vi "FuncVI-viRun.vi"(5 "InstanceRef":T2, 9 "arg list":T1[](array[typedef]) {"num" format="%.2f"}) -> (0 "error out":bool, 3 "result":T1 {"num" format="%.2f"})   [LabVIEW 2021]
doc: "::: CalcExpress Toolkit :::\nCopyright (c) 2000-2026 Konstantin Shifershteyn. All rights reserved."
uses:
  cetypes.llb/CalcExpress Function Argument Info.ctl
  cetypes.llb/CalcExpress Instance RefNum.ctl
panel:
  in  "max arg num":i32=1000
  in  "min arg num":i32=1
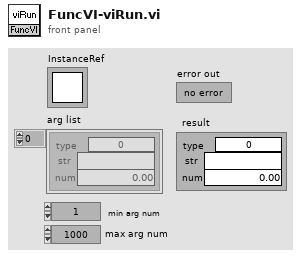
[diagram p1: front panel]
types:
  T1 = typedef "CalcExpress Function Argument Info.ctl" = cluster{"type":u32, "str":string, "num":dbl}
  T2 = typedef "CalcExpress Instance RefNum.ctl" = refnum<k1>
  T3 = enum32{"String", "DBL Number", "identifier", "1D Array of DBL", "2D Array of DBL", "CDB Number", "1D Array of CDB", "2D Array of CDB", "1D Array of String", "2D Array of String", "Unknown data type"}
  T4 = cluster{"index":i32, "data type":enum32{"String", "DBL Number", "identifier", "1D Array of DBL", "2D Array of DBL", "CDB Number", "1D Array of CDB", "2D Array of CDB", "1D Array of String", "2D Array of String", "Unknown data type"}, "default num":dbl, "default str":string}[]
  T5 = cluster{"use this constant to specify a predefined type":enum32{"String", "DBL Number", "identifier", "1D Array of DBL", "2D Array of DBL", "CDB Number", "1D Array of CDB", "2D Array of CDB", "1D Array of String", "2D Array of String", "Unknown data type"}, string, "code":i32}
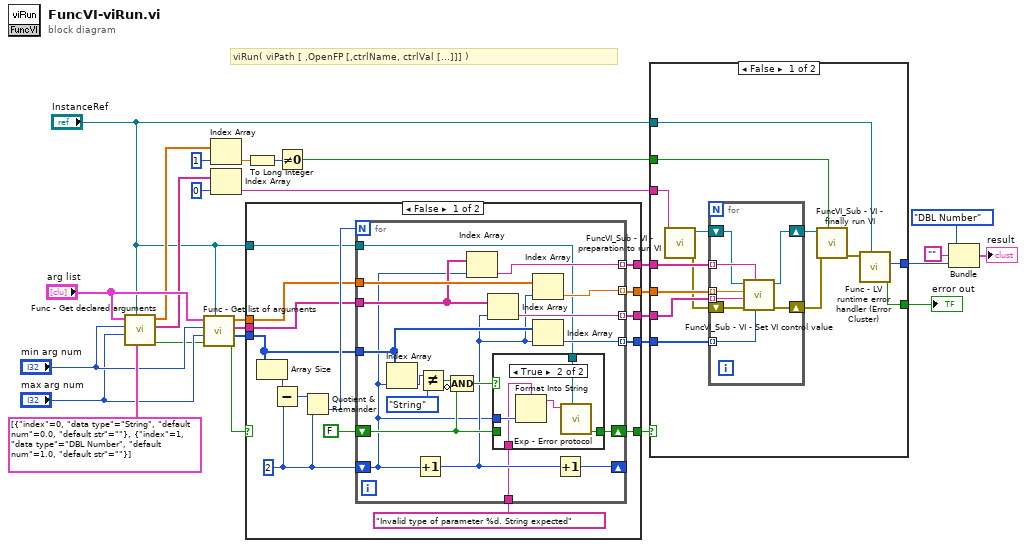
[diagram p0: block diagram]
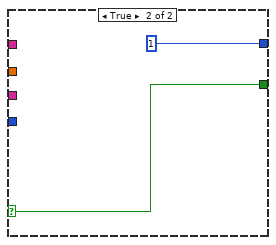
[diagram p2: hidden frame]
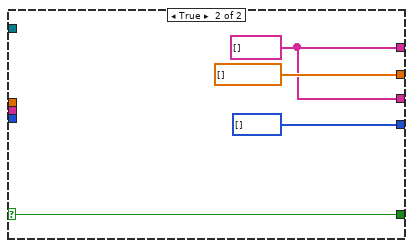
[diagram p4: hidden frame]
diagram:
  # "viRun( viPath [ ,OpenFP [,ctrlName, ctrlVal [...]]] )"
  n1 = call "Func - Get declared arguments.vi"("arg descriptors"=T4 [{"index"=0, "data type"=enum."String", "default num"=0.0, "default str"=""}, {"index"=1, "data type"=enum."DBL Number", "default num"=1.0, "default str"=""}] ("args descriptors"), "InstanceRef"="InstanceRef", "max arg num"="max arg num", "min arg num"="min arg num", "arg list"="arg list") -> ("error out"=w20:bool, "str list"=w16:string[], "num list"=w17:dbl[])  [unwired: 3 in, 1 out]
  n2 = call "Func - Get list of arguments.vi"("InstanceRef"="InstanceRef", "error in"=w20, "max arg num"="max arg num", "min arg num"="min arg num", "arg list"="arg list") -> ("error out"=w28:bool, "type list"=w25:u32[], "str list"=w26:string[], "num list"=w27:dbl[])  [unwired: 3 in]
  n3 = Index Array(array=w17, index=1) -> (element=w13:dbl)
  n4 = Index Array(array=w16, index=0) -> (element=w1:string)
  n5 = case shown="False" w28 {
    selector: w28 -> [_ w71]
    tunnel: [w34 w71] -> w14
    tunnel: w27 -> [w37 _]
    tunnel: w26 -> [w36 _]
    tunnel: w25 -> [w38 _]
    tunnel: [w33 dbl[] []] -> w12
    tunnel: [w32 w68] -> w11
    tunnel: [w31 u32[] []] -> w10
    tunnel: [w30 w68] -> w9
    tunnel: "InstanceRef" -> [w29 _]
    frame False {
      w40 = 2 ("y")
      n6 = Array Size(array=w38) -> (size(s)=w43:i32)
      n7 = Subtract(x=w43, y=w40) -> (x-y=w42:i32)
      n8 = Quotient & Remainder(x=w42, y=w40) -> (floor(x/y)=w41:i32)  [unwired: 1 out]
      n9 = for {
        N: w41 -> [_]
        shift-right: [w61] -> _
        shift-left: w40 -> [w45]
        shift-right: [w60] -> w34
        shift-left: FALSE -> [w56]
        tunnel: w38 -> [w53]
        tunnel: w37 -> [w54]
        tunnel: w36 -> [w49]
        tunnel: [w52] -> w31 mode=indexing
        tunnel: [w51] -> w32 mode=indexing
        tunnel: [w50] -> w33 mode=indexing
        tunnel: [w47] -> w30 mode=indexing
        tunnel: "Invalid type of parameter %d. String expected" -> [w46]
        tunnel: w29 -> [w44]
        n10 = Index Array(array=w53, index=w45) -> (element=w59:u32)
        n11 = Increment(x=w45) -> (x+1=w48:i32)
        n12 = Not Equal?(x=w59, y=T3."String") -> (x != y?=w57:bool)
        n13 = Compound Arithmetic op=AND(w57, invert w56) -> (w55:bool)
        n14 = Index Array(array=w49, index=w45) -> (element=w47:string)
        n15 = Index Array(array=w49, index=w48) -> (element=w51:string)
        n16 = case shown="True" w55 {
          tunnel: [w62 w67] -> w60
          tunnel: w56 -> [w62 _]
          tunnel: w45 -> [_ w65]
          tunnel: w46 -> [_ w64]
          tunnel: w44 -> [_ w63]
          frame False {
          }
          frame True {
            n17 = Format Into String(format string=w64, w65) -> (resulting string=w66:string)  [unwired: 2 in, 1 out]
            n18 = call "Exp - Error protocol.vi"("InstanceRef"=w63, "error message in"=w66) -> ("error out"=w67:bool)  [unwired: 6 in, 1 out]
          }
        }
        n19 = Index Array(array=w54, index=w48) -> (element=w50:dbl)
        n20 = Index Array(array=w53, index=w48) -> (element=w52:u32)
        n21 = Increment(x=w48) -> (x+1=w61:i32)
      }
    }
    frame True {
      w68 = string[] []
    }
  }
  n22 = To Long Integer(number=w13) -> (32bit integer=w15:i32)
  n23 = Not Equal To 0?(x=w15) -> (x != 0?=w8:bool)
  n24 = case shown="False" w14 {
    selector: w14 -> [_ w95]
    tunnel: w12 -> [w85 _]
    tunnel: w11 -> [w84 _]
    tunnel: w10 -> [w83 _]
    tunnel: w9 -> [w82 _]
    tunnel: w1 -> [w79 _]
    tunnel: w8 -> [w77 _]
    tunnel: [w72 w95] -> w6
    tunnel: "InstanceRef" -> [w74 _]
    tunnel: [w73 1 ("code")] -> w3
    frame False {
      n25 = call "FuncVI_Sub - VI - preparation to run VI.vi"("VI name or path"=w79) -> ("error out"=w80:errorcluster, "VI Refnum"=w81:refnum<vi>)  [unwired: 8 in, 1 out]
      n26 = for {
        tunnel: w85 -> [w93] mode=indexing
        tunnel: w84 -> [w92] mode=indexing
        tunnel: w83 -> [w91] mode=indexing
        tunnel: w82 -> [w90] mode=indexing
        shift-right: [w88] -> w76
        shift-left: w80 -> [w89]
        shift-right: [w87] -> w78
        shift-left: w81 -> [w86]
        n27 = call "FuncVI_Sub - VI - Set VI control value.vi"("type"=w91, "control name"=w90, "error in"=w89, "str"=w92, "dbl"=w93, "VI Ref"=w86) -> ("error out"=w88:errorcluster, "dup VI Ref"=w87:refnum<vi>)  [unwired: 4 in]
      }
      n28 = call "FuncVI_Sub - VI - finally run VI.vi"("open FP"=w77, "error in"=w76, "vi RefNum"=w78) -> ("error out"=w75:errorcluster)  [unwired: 8 in]
      n29 = call "Func - LV runtime error handler (Error Cluster).vi"("InstanceRef"=w74, "LabVIEW error"=w75) -> ("error out"=w72:bool, "LV error code"=w73:i32)  [unwired: 4 in, 2 out]
    }
    frame True {
    }
  }
  "error out" <- w6
  n30 = Bundle("use this constant to specify a predefined type"=T3."DBL Number", "", "code"=w3) -> (→"result":T5)  [unwired: 1 in]
